vi "Add Remove Test.vi"() -> (0 "error out":errorcluster, 1 "deleted line name?":bool, 2 "channel deleted?":bool, 3 "channel added?":bool)   [LabVIEW 2014, in "Shared Memory tests.lvlib"]
doc: "Tests the Add Line and Remove Line functions."
uses:
  Shared Memory tests.lvlib
  <vilib>/NI/Tag Bus/tag/Data Type.ctl
  module/configuration/Line.ctl
  <vilib>/NI/Tag Bus Module Framework/channel/TBM channel.lvclass
  <vilib>/NI/Tag Bus Module Framework/channel/channel classification.ctl
  module/configuration/Shared Memory configuration.lvclass
  <vilib>/NI/Tag Bus/tag/tag descriptor.lvclass
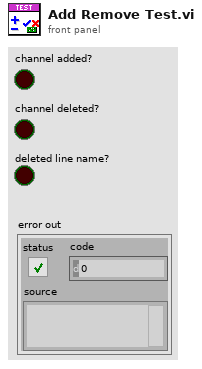
[diagram p1: front panel]
types:
  T1 = typedef "TBM channel.lvclass/channel classification.ctl" = enum16{"input data", "output data", "processing parameter", "processing result"}
  T2 = typedef "Shared Memory configuration.lvclass/Line.ctl" = cluster{"channel":refnum<class "TBM channel.lvclass">}
  T3 = typedef "tag bus.lvlib/tag descriptor.lvclass/Data Type.ctl" = enum16{"Double", "Single", "I64", "I32", "I16", "I8", "U64", "U32", "U16", "U8", "Boolean", "String", "Array of Double", "Array of Single", "Array of I64", "Array of I32", "Array of I16", "Array of I8", "Array of U64", "Array of U32", "Array of U16", "Array of U8", "Array of Boolean", "Array of String"}
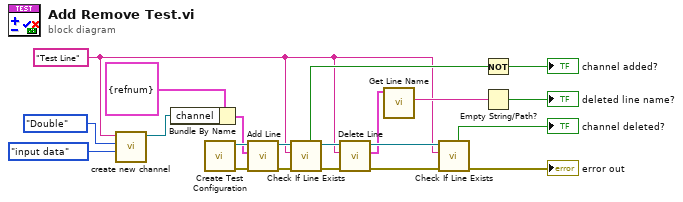
[diagram p0: block diagram]
diagram:
  w5 = "Test Line" ("channel name")
  n1 = call <vilib>:"create new channel.vi"("channel classification"=channel_classification."input data", "data type"=Data_Type."Double", "channel name"=w5) -> ("channel"=w20:refnum<class "TBM channel.lvclass">)  [unwired: 8 in]
  n2 = Bundle By Name(cluster=T2 {"channel"=refnum} ("Line"), "channel"=w20) -> (w18:T2)
  n3 = call "Create Test Configuration.vi"() -> ("error out"=w11:errorcluster, "Module Configuration"=w21:refnum<class "Shared Memory configuration.lvclass">)  [unwired: 3 in, 7 out]
  n4 = call "Add Line.vi"("error in"=w11, "Line"=w18, "Shared Memory configuration in"=w21) -> ("error out"=w13:errorcluster, "Shared Memory configuration out"=w16:refnum<class "Shared Memory configuration.lvclass">)  [unwired: 6 in, 1 out]
  n5 = call-dynamic "Check If Line Exists.vi"("error in"=w13, "Name to Locate"=w5, "Shared Memory configuration in"=w16) -> ("error out"=w12:errorcluster, "Shared Memory configuration out"=w15:refnum<class "Shared Memory configuration.lvclass">, "Found?"=w14:bool)  [unwired: 4 in, 2 out]
  n6 = call "Delete Line.vi"("error in"=w12, "Line Name"=w5, "Shared Memory configuration in"=w15) -> ("error out"=w10:errorcluster, "Deleted Line"=w7:T2, "Shared Memory configuration out"=w8:refnum<class "Shared Memory configuration.lvclass">)  [unwired: 6 in]
  n7 = call "Get Line Name.vi"("Line in"=w7) -> ("Name"=w6:string)  [unwired: 8 in, 2 out]
  n8 = call-dynamic "Check If Line Exists.vi"("error in"=w10, "Name to Locate"=w5, "Shared Memory configuration in"=w8) -> ("error out"=→"error out":errorcluster, "Found?"=→"channel deleted?":bool)  [unwired: 4 in, 3 out]
  n9 = Not(x=w14) -> (.not. x?=→"channel added?":bool)
  n10 = Empty String/Path?(string/path=w6) -> (empty?=→"deleted line name?":bool)
